vi "Stop Acq.vi"(8 "error in (no error)":errorcluster, 11 "HamamatsuFluor in":refnum<class "HamamatsuFluor.lvclass">) -> (0 "error out":errorcluster, 3 "HamamatsuFluor out":refnum<class "HamamatsuFluor.lvclass">)   [LabVIEW 2020, in "DAQ Timed SPIM.lvlib" / "HamamatsuFluor_v2.lvlib" / "HamamatsuFluor.lvclass"]
uses:
  HamamatsuFluor.lvclass
  HamamatsuFluor.lvclass/HamamatsuFluor.ctl
  Abstract DAQ Triggered Actor/Abstract DAQ Triggered Actor.lvclass
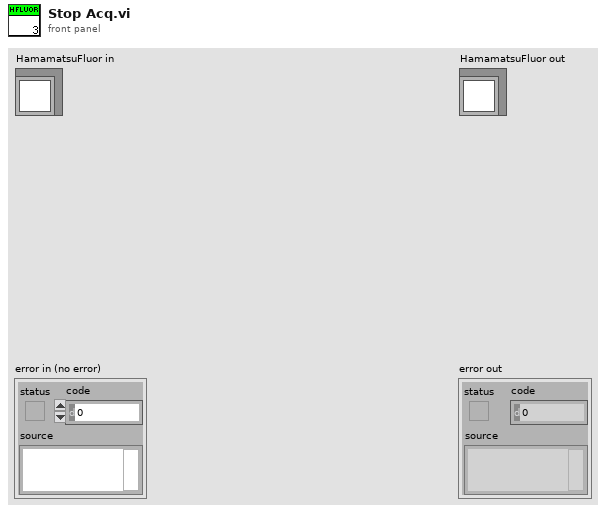
[diagram p1: front panel]
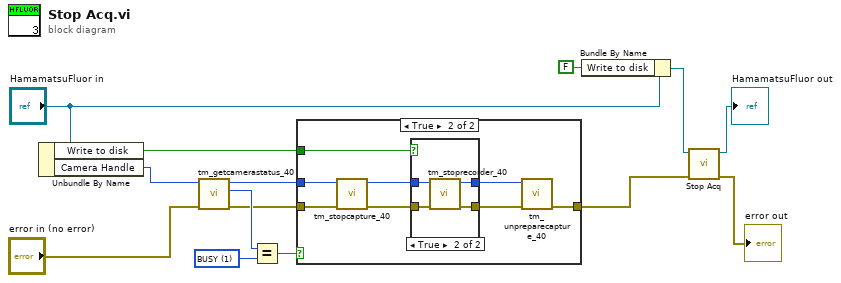
[diagram p0: block diagram]
diagram:
  w7 = 1 items=["ERROR", "BUSY", "READY", "STABLE", "UNSTABLE"] ("Status")
  n1 = Unbundle By Name("HamamatsuFluor in") -> ("Write to disk"=w6:bool, "Camera Handle"=w5:u32)
  n2 = call <userlib>:"tm_getcamerastatus_40.vi"("error in (no error)"="error in (no error)", "Handle in"=w5) -> ("error out"=w3:errorcluster, "Status"=w8:i32, "Handle out"=w2:u32)  [unwired: 7 in]
  n3 = Equal?(x=w8, y=w7) -> (x = y?=w1:bool)
  n4 = case shown="True" w1 {
    tunnel: [w15 w19] -> w12
    tunnel: w6 -> [_ w18]
    tunnel: w3 -> [w15 w17]
    tunnel: w2 -> [_ w16]
    frame False {
    }
    frame True {
      n5 = call <userlib>:"tm_stopcapture_40.vi"("error in (no error)"=w17, "Handle in"=w16) -> ("error out"=w22:errorcluster, "Handle out"=w23:u32)  [unwired: 8 in]
      n6 = case shown="True" w18 {
        tunnel: [w25 w29] -> w21
        tunnel: [w24 w28] -> w20
        tunnel: w23 -> [w25 w27]
        tunnel: w22 -> [w24 w26]
        frame False {
        }
        frame True {
          n7 = call <userlib>:"tm_stoprecorder_40.vi"("error in (no error)"=w26, "Handle in"=w27) -> ("error out"=w28:errorcluster, "Handle out"=w29:u32)  [unwired: 8 in]
        }
      }
      n8 = call <userlib>:"tm_unpreparecapture_40.vi"("error in (no error)"=w20, "Handle in"=w21) -> ("error out"=w19:errorcluster)  [unwired: 8 in, 1 out]
    }
  }
  n9 = Bundle By Name(cluster="HamamatsuFluor in", "Write to disk"=FALSE) -> (w10:refnum<class "HamamatsuFluor.lvclass">)
  n10 = call-parent "Stop Acq.vi"("error in (no error)"=w12, "Abstract Camera Actor in"=w10) -> ("error out"=→"error out":errorcluster, "Abstract Camera Actor out"=→"HamamatsuFluor out":refnum<class "HamamatsuFluor.lvclass">)  [unwired: 8 in]
